vi "Shell_exec.vi"() -> (0 "Firmware Instalado":bool, 1 "return code":i32, 3 "standard output":string)   [LabVIEW 2026]
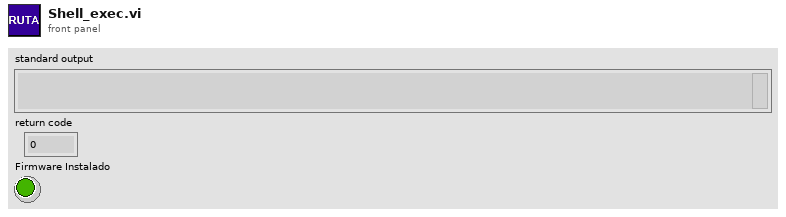
[diagram p1: front panel]
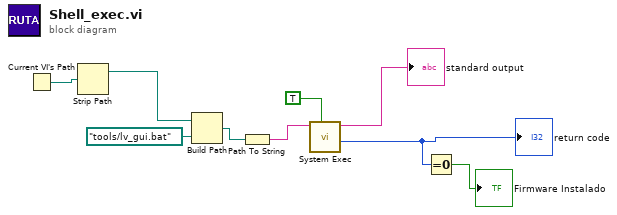
[diagram p0: block diagram]
diagram:
  n1 = Current VI's Path() -> (path=w3:path)
  n2 = Strip Path(path=w3) -> (stripped path=w4:path)  [unwired: 1 out]
  n3 = Build Path(base path=w4, name or relative path=path "tools/lv_gui.bat") -> (appended path=w5:path)
  n4 = Path To String(path=w5) -> (string=w6:string)
  n5 = call <vilib>:"System Exec.vi"("wait until completion? (T)"=TRUE, "command line"=w6) -> ("return code"=w8:i32, "standard output"=→"standard output":string)  [unwired: 6 in, 2 out]
  "return code" <- w8
  n6 = Equal To 0?(x=w8) -> (x = 0?=→"Firmware Instalado":bool)
